vi "Sapphire488GUI.vi"() -> ()   [LabVIEW 2017]
doc: "Use this template to build a user interface event handler design pattern. Use this pattern for dialog boxes and other user interfaces. You also can create and execute user-defined events that the VI can handle the same way as user interface events."
uses:
  states/488intStates.ctl
  states/488GUIStates.ctl
  <vilib>/Utility/config.llb/Read Key (String).vi
  <vilib>/Instr/_visa.llb/VISA Configure Serial Port (Instr).vi
  <vilib>/Utility/config.llb/Write Key (String).vi
  <vilib>/Utility/config.llb/NI_LVConfig.lvlib
panel:
  in  "488_High":bool
  in  "488_Low":bool
  out "Controller T":string
  out "Fault":string
  out "Diode Temp":string
  out "BasePlate T":string
  in  "SetPower [mW]":u8(slide)=20 min=20 scale=0.0..1.0
  in  "stop":bool
  out "PowesSupplyHours":string
  out "HeadHours":string
  out "Power [mW]":dbl(knob) scale=0.0..1.0
  out "?":T1
  out "Key":bool
  out "NomLP":string
  out "MaxLP":string
  out "MinLP":string
  out "Name":string
  in  "ComPort":refnum<visa-resource-name>
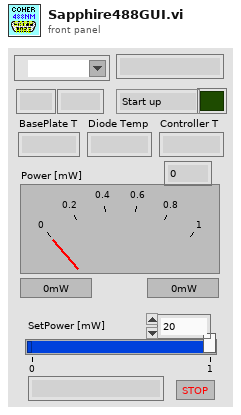
[diagram p1: front panel]
types:
  T1 = typedef "488intStates.ctl" = enum16{"Start up", "Warmup", "Standby", "Laser on", "Laser ready", "Fault"}
  T2 = typedef "488GUIStates.ctl" = enum16{"init", "startup", "idle", "stop"}
  T3 = typedef "NI_LVConfig.lvlib/Config Data RefNum.ctl" = refnum<k1>
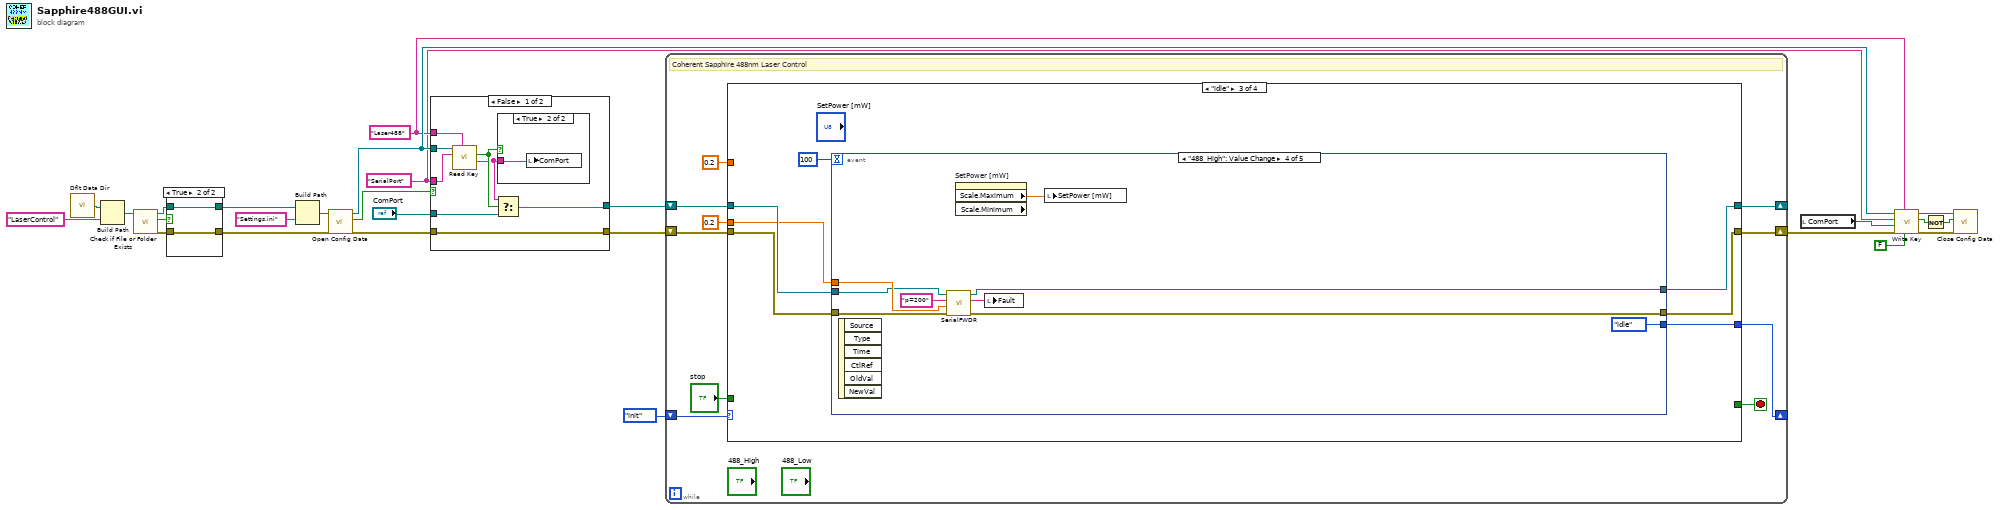
[diagram p0: block diagram]
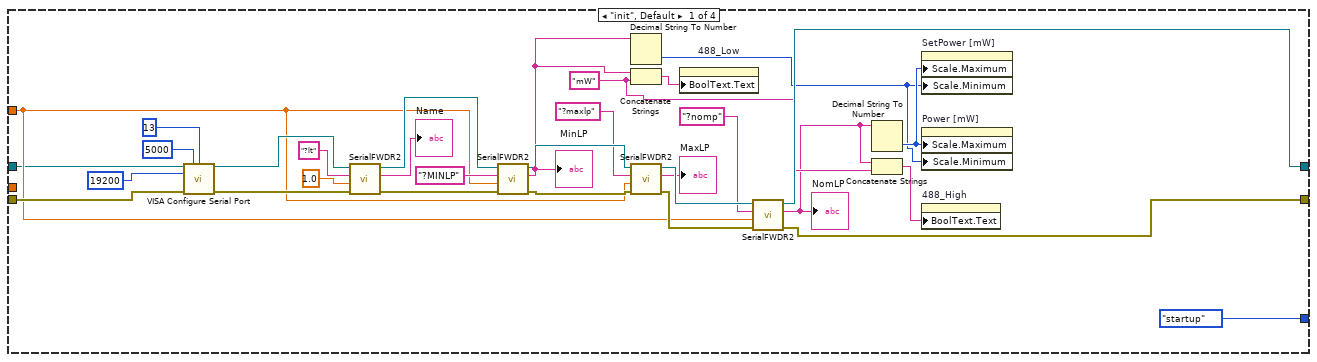
[diagram p2: hidden frame]
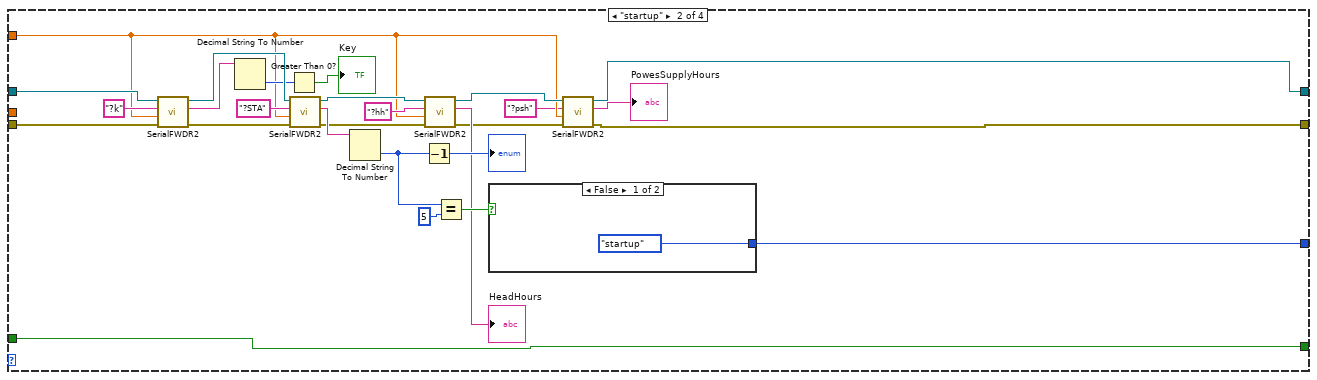
[diagram p3: hidden frame]
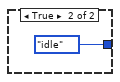
[diagram p4: hidden frame]
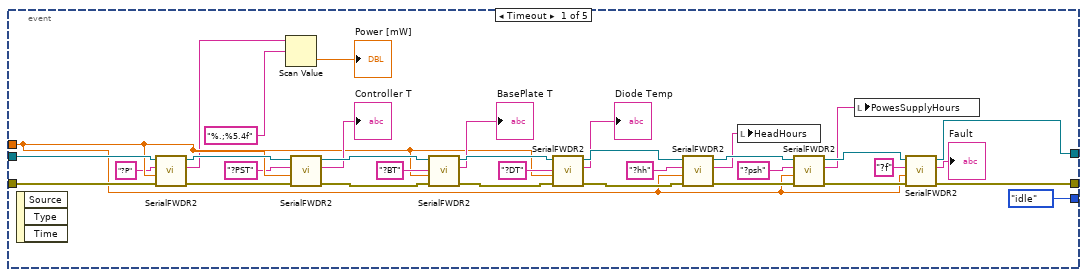
[diagram p5: hidden frame]
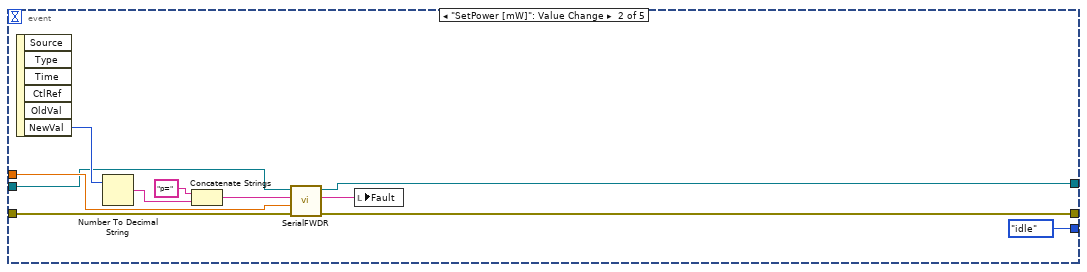
[diagram p6: hidden frame]
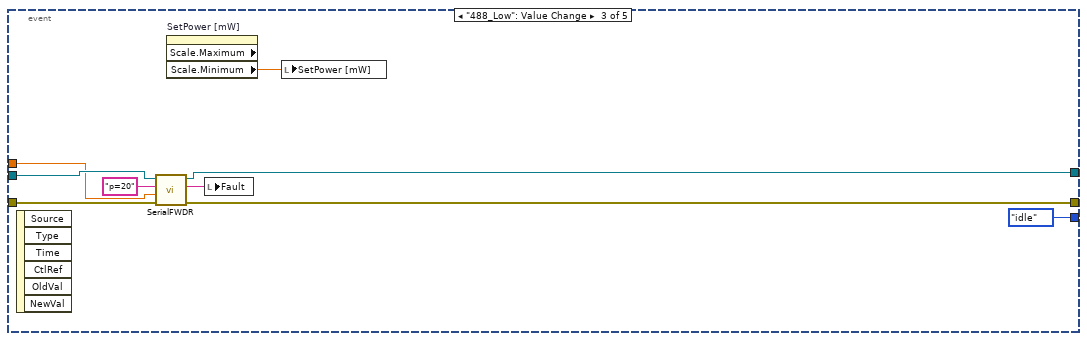
[diagram p7: hidden frame]
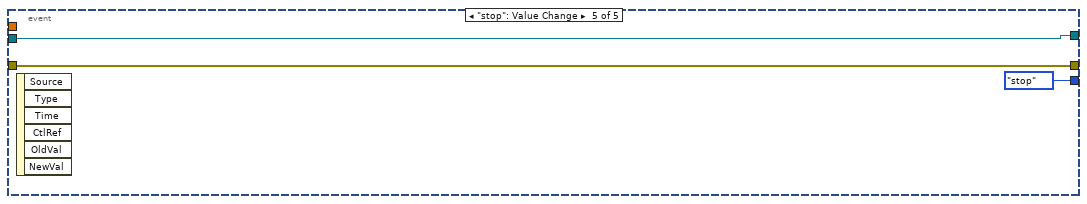
[diagram p8: hidden frame]
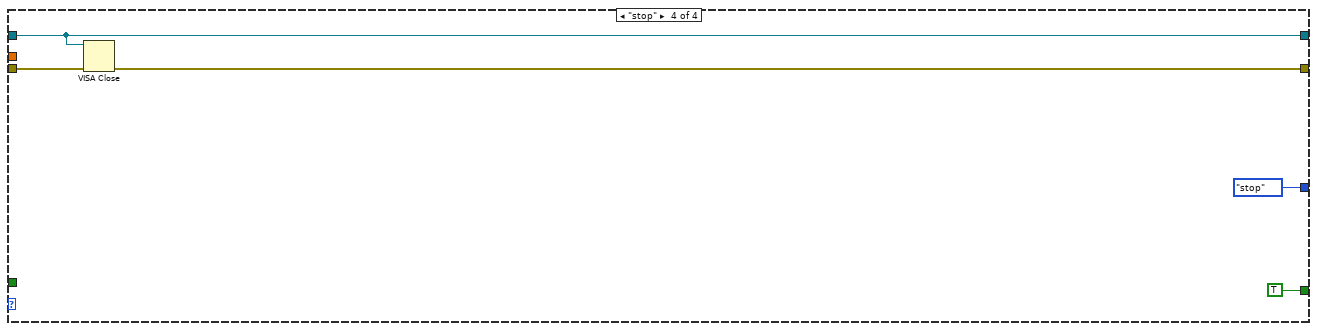
[diagram p9: hidden frame]
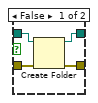
[diagram p12: hidden frame]
diagram:
  w5 = "SerialPort" ("key")
  w6 = "Laser488" ("section")
  n1 = call <vilib>:"Dflt Data Dir.vi"() -> ("App:Default Data Directory"=w22:path)
  n2 = Build Path(base path=w22, name or relative path="LaserControl") -> (appended path=w19:path)
  n3 = call <vilib>:"Check if File or Folder Exists.vi"("path"=w19) -> ("error out"=w16:errorcluster, "file or folder exists?"=w18:bool, "dup path"=w17:path)  [unwired: 8 in]
  n4 = case shown="True" w18 {
    tunnel: [w29 w32] -> w14
    tunnel: w17 -> [w30 w32]
    tunnel: w16 -> [w28 w31]
    tunnel: [w27 w31] -> w15
    frame False {
      n5 = Create Folder(path (use dialog)=w30, error in=w28) -> (created path=w29:path, error out=w27:errorcluster)  [unwired: 1 in, 1 out]
    }
    frame True {
    }
  }
  n6 = Build Path(base path=w14, name or relative path="Settings.ini") -> (appended path=w20:path)
  n7 = call <vilib>:"Open Config Data.vi"("error in (no error)"=w15, "configuration file path"=w20) -> ("error out"=w12:errorcluster, "file created?"=w9:bool, "refnum"=w10:T3)  [unwired: 7 in]
  n8 = case shown="False" w9 {
    tunnel: "ComPort" -> [w37 w43]
    tunnel: w12 -> [w36 w42]
    tunnel: w10 -> [w38 _]
    tunnel: [w36 w42] -> w3
    tunnel: [w35 w43] -> w2
    tunnel: w6 -> [w34 _]
    tunnel: w5 -> [w33 _]
    frame False {
      n9 = call-poly <vilib>:"Read Key.vi"("section"=w34, "key"=w33, "refnum"=w38) -> ("value"=w39:string, "found?"=w40:bool)  [unwired: 5 in, 2 out]
      n10 = Select(t=w39, s=w40, f=w37) -> (s? t:f=w35:string)
      n11 = case shown="True" w40 {
        tunnel: w39 -> [_ w41]
        frame False {
        }
        frame True {
          n12 = local write "ComPort"(w41) -> ()
        }
      }
    }
    frame True {
    }
  }
  n13 = while {
    shift-right: [w52] -> _
    shift-left: 488GUIStates."init" -> [w53]
    shift-right: [w49] -> _
    shift-left: w2 -> [w48]
    shift-right: [w47] -> w1
    shift-left: w3 -> [w51]
    stop <- w46 stop-if-true
    # "Coherent Sapphire 488nm Laser Control"
    n14 = case shown="\"idle\"" w53 {
      tunnel: [488GUIStates."startup" w98 w120 488GUIStates."stop"] -> w52
      tunnel: w51 -> [w66 w111 w116 w190]
      tunnel: [w65 w89 w117 w189] -> w47
      tunnel: 0.2 ("Delay Time (s)") -> [w64 w88 _ _]
      tunnel: [w63 w91 w119 w188] -> w49
      tunnel: w48 -> [w62 w110 w118 w188]
      tunnel: [_ w85 _ TRUE] -> w46
      tunnel: "stop" -> [_ w85 _ _]
      tunnel: 0.2 ("Delay Time (s)") -> [_ _ w114 _]
      frame "init", Default {
        w58 = "mW" ("string")
        n15 = call-poly "VISA Configure Serial Port"("VISA resource name"=w62, "timeout (10sec)"=u32 5000, "termination char\n(0xA = '\\n' = LF)"=u8 13 ("termination char\n(0xA = '\\n' = LF)"), "baud rate (9600)"=u32 19200, "error in (no error)"=w66) -> ("VISA resource name out"=w77:refnum<visa-resource-name>, "error out"=w76:errorcluster)  [unwired: 9 in]
        n16 = call "SerialFWDR2.vi"("error in (no error)"=w76, "Delay Time (s)"=1.0, "CommandString"="?lt", "VISA Refnum in"=w77) -> ("error out"=w73:errorcluster, "trimmed string"=→"Name":string, "VISA Refnum out"=w75:refnum<visa-resource-name>)  [unwired: 5 in]
        n17 = call "SerialFWDR2.vi"("error in (no error)"=w73, "Delay Time (s)"=w64, "CommandString"="?MINLP", "VISA Refnum in"=w75) -> ("error out"=w72:errorcluster, "trimmed string"=w55:string, "VISA Refnum out"=w74:refnum<visa-resource-name>)  [unwired: 5 in]
        "MinLP" <- w55
        n18 = Decimal String To Number(string=w55) -> (number=w56:i32)  [unwired: 2 in, 1 out]
        n19 = Concatenate Strings(w55, w58) -> (w60:string)
        n20 = call "SerialFWDR2.vi"("error in (no error)"=w72, "Delay Time (s)"=w64, "CommandString"="?maxlp", "VISA Refnum in"=w74) -> ("error out"=w70:errorcluster, "trimmed string"=→"MaxLP":string, "VISA Refnum out"=w71:refnum<visa-resource-name>)  [unwired: 5 in]
        n21 = property on="488_Low" class="Bool"("BoolText.Text"=w60) -> ()  [unwired: 2 in, 2 out]
        n22 = call "SerialFWDR2.vi"("error in (no error)"=w70, "Delay Time (s)"=w64, "CommandString"="?nomp", "VISA Refnum in"=w71) -> ("error out"=w65:errorcluster, "trimmed string"=w54:string, "VISA Refnum out"=w63:refnum<visa-resource-name>)  [unwired: 5 in]
        "NomLP" <- w54
        n23 = Decimal String To Number(string=w54) -> (number=w57:i32)  [unwired: 2 in, 1 out]
        n24 = Concatenate Strings(w54, w58) -> (w59:string)
        n25 = property on="SetPower [mW]" class="Slide (strict)"("Scale.Maximum"=w57, "Scale.Minimum"=w56) -> ()  [unwired: 2 in, 2 out]
        n26 = property on="Power [mW]" class="Knob (strict)"("Scale.Maximum"=w57, "Scale.Minimum"=w56) -> ()  [unwired: 2 in, 2 out]
        n27 = property on="488_High" class="Bool"("BoolText.Text"=w59) -> ()  [unwired: 2 in, 2 out]
      }
      frame "startup" {
        n28 = call "SerialFWDR2.vi"("error in (no error)"=w111, "Delay Time (s)"=w88, "CommandString"="?k", "VISA Refnum in"=w110) -> ("error out"=w106:errorcluster, "trimmed string"=w107:string, "VISA Refnum out"=w105:refnum<visa-resource-name>)  [unwired: 5 in]
        n29 = Decimal String To Number(string=w107) -> (number=w97:i32)  [unwired: 2 in, 1 out]
        n30 = Greater Than 0?(x=w97) -> (x > 0?=→"Key":bool)
        n31 = call "SerialFWDR2.vi"("error in (no error)"=w106, "Delay Time (s)"=w88, "CommandString"="?STA", "VISA Refnum in"=w105) -> ("error out"=w95:errorcluster, "trimmed string"=w103:string, "VISA Refnum out"=w96:refnum<visa-resource-name>)  [unwired: 5 in]
        n32 = Decimal String To Number(string=w103) -> (number=w100:i32)  [unwired: 2 in, 1 out]
        n33 = Decrement(x=w100) -> (x-1=→"?":i32)
        n34 = call "SerialFWDR2.vi"("error in (no error)"=w95, "Delay Time (s)"=w88, "CommandString"="?hh", "VISA Refnum in"=w96) -> ("error out"=w90:errorcluster, "trimmed string"=→"HeadHours":string, "VISA Refnum out"=w92:refnum<visa-resource-name>)  [unwired: 5 in]
        n35 = Equal?(x=w100, y=5) -> (x = y?=w99:bool)
        n36 = case shown="False" w99 {
          tunnel: [488GUIStates."startup" 488GUIStates."idle"] -> w98
          frame False {
          }
          frame True {
          }
        }
        n37 = call "SerialFWDR2.vi"("error in (no error)"=w90, "Delay Time (s)"=w88, "CommandString"="?psh", "VISA Refnum in"=w92) -> ("error out"=w89:errorcluster, "trimmed string"=→"PowesSupplyHours":string, "VISA Refnum out"=w91:refnum<visa-resource-name>)  [unwired: 5 in]
      }
      frame "idle" {
        n38 = event shown="[3] \"488_High\": Value Change" {
          selector: _ -> [_ _ _ _ _]
          dyn-events: _ -> [_ _ _ _ _]
          timeout: 100 -> [_ _ _ _ _]
          tunnel: [488GUIStates."idle" 488GUIStates."idle" 488GUIStates."idle" 488GUIStates."idle" 488GUIStates."stop"] -> w120
          tunnel: [w121 w156 w171 w179 w185] -> w119
          tunnel: w118 -> [w130 w157 w170 w176 w185]
          tunnel: [w122 w160 w172 w181 w184] -> w117
          tunnel: w116 -> [w129 w161 w173 w182 w184]
          tunnel: w114 -> [w128 w159 w167 w177 _]
          event Timeout {
            n39 = event-data() -> ()  [unwired: 1 in, 3 out]
            n40 = call "SerialFWDR2.vi"("error in (no error)"=w129, "Delay Time (s)"=w128, "CommandString"="?P", "VISA Refnum in"=w130) -> ("error out"=w131:errorcluster, "trimmed string"=w124:string, "VISA Refnum out"=w132:refnum<visa-resource-name>)  [unwired: 5 in]
            n41 = Scan Value(string=w124, format string="%.;%5.4f") -> (value=→"Power [mW]":dbl)  [unwired: 1 in, 1 out]
            n42 = call "SerialFWDR2.vi"("error in (no error)"=w131, "Delay Time (s)"=w128, "CommandString"="?PST", "VISA Refnum in"=w132) -> ("error out"=w134:errorcluster, "trimmed string"=→"Controller T":string, "VISA Refnum out"=w135:refnum<visa-resource-name>)  [unwired: 5 in]
            n43 = call "SerialFWDR2.vi"("error in (no error)"=w134, "Delay Time (s)"=w128, "CommandString"="?BT", "VISA Refnum in"=w135) -> ("error out"=w149:errorcluster, "trimmed string"=→"BasePlate T":string, "VISA Refnum out"=w153:refnum<visa-resource-name>)  [unwired: 5 in]
            n44 = call "SerialFWDR2.vi"("error in (no error)"=w149, "Delay Time (s)"=w128, "CommandString"="?DT", "VISA Refnum in"=w153) -> ("error out"=w148:errorcluster, "trimmed string"=→"Diode Temp":string, "VISA Refnum out"=w152:refnum<visa-resource-name>)  [unwired: 5 in]
            n45 = call "SerialFWDR2.vi"("error in (no error)"=w148, "Delay Time (s)"=w128, "CommandString"="?hh", "VISA Refnum in"=w152) -> ("error out"=w147:errorcluster, "trimmed string"=w140:string, "VISA Refnum out"=w151:refnum<visa-resource-name>)  [unwired: 5 in]
            n46 = local write "HeadHours"(w140) -> ()
            n47 = call "SerialFWDR2.vi"("error in (no error)"=w147, "Delay Time (s)"=w128, "CommandString"="?psh", "VISA Refnum in"=w151) -> ("error out"=w146:errorcluster, "trimmed string"=w138:string, "VISA Refnum out"=w150:refnum<visa-resource-name>)  [unwired: 5 in]
            n48 = local write "PowesSupplyHours"(w138) -> ()
            n49 = call "SerialFWDR2.vi"("error in (no error)"=w146, "Delay Time (s)"=w128, "CommandString"="?f", "VISA Refnum in"=w150) -> ("error out"=w122:errorcluster, "trimmed string"=→"Fault":string, "VISA Refnum out"=w121:refnum<visa-resource-name>)  [unwired: 5 in]
          }
          event "SetPower [mW]": Value Change {
            n50 = event-data() -> ("NewVal"=w164:u8)  [unwired: 1 in, 5 out]
            n51 = Number To Decimal String(number=w164) -> (decimal integer string=w163:string)  [unwired: 1 in]
            n52 = Concatenate Strings("p=", w163) -> (w158:string)
            n53 = call "SerialFWDR.vi"("error in (no error)"=w161, "Delay Time (s)"=w159, "CommandString"=w158, "VISA Refnum in"=w157) -> ("error out"=w160:errorcluster, "trimmed string"=w155:string, "VISA Refnum out"=w156:refnum<visa-resource-name>)  [unwired: 5 in]
            n54 = local write "Fault"(w155) -> ()
          }
          event "488_Low": Value Change {
            n55 = event-data() -> ()  [unwired: 1 in, 6 out]
            n56 = call "SerialFWDR.vi"("error in (no error)"=w173, "Delay Time (s)"=w167, "CommandString"="p=20", "VISA Refnum in"=w170) -> ("error out"=w172:errorcluster, "trimmed string"=w169:string, "VISA Refnum out"=w171:refnum<visa-resource-name>)  [unwired: 5 in]
            n57 = property on="SetPower [mW]" class="Slide (strict)" props=["Scale", "Maximum", "Scale", "Minimum"]() -> ("Scale.Minimum"=w166:dbl)  [unwired: 2 in, 3 out]
            n58 = local write "Fault"(w169) -> ()
            n59 = local write "SetPower [mW]"(w166) -> ()
          }
          event "488_High": Value Change {
            n60 = event-data() -> ()  [unwired: 1 in, 6 out]
            n61 = call "SerialFWDR.vi"("error in (no error)"=w182, "Delay Time (s)"=w177, "CommandString"="p=200", "VISA Refnum in"=w176) -> ("error out"=w181:errorcluster, "trimmed string"=w180:string, "VISA Refnum out"=w179:refnum<visa-resource-name>)  [unwired: 5 in]
            n62 = property on="SetPower [mW]" class="Slide (strict)" props=["Scale", "Maximum", "Scale", "Minimum"]() -> ("Scale.Maximum"=w175:dbl)  [unwired: 2 in, 3 out]
            n63 = local write "Fault"(w180) -> ()
            n64 = local write "SetPower [mW]"(w175) -> ()
          }
          event "stop": Value Change {
            n65 = event-data() -> ()  [unwired: 1 in, 6 out]
          }
        }
      }
      frame "stop" {
        n66 = VISA Close(VISA resource name=w188, error in (no error)=w190) -> (error out=w189:errorcluster)
      }
    }
  }
  n67 = local read "ComPort"() -> (w25:refnum<visa-resource-name>)
  n68 = call-poly <vilib>:"Write Key.vi"("write raw string? (F)"=FALSE, "section"=w6, "error in (no error)"=w1, "value"=w25, "key"=w5, "refnum"=w10) -> ("error out"=w23:errorcluster, "found?"=w8:bool, "refnum out"=w24:T3)  [unwired: 3 in]
  n69 = Not(x=w8) -> (.not. x?=w7:bool)
  n70 = call <vilib>:"Close Config Data.vi"("error in (no error)"=w23, "write file if changed (T)"=w7, "refnum"=w24) -> ()  [unwired: 7 in, 2 out]
